vi "RDC-tools-generate_temp_array.vi"(7 "Increment":dbl=0.1, 11 "temp Cx10":dbl[](array[numeric])) -> (3 "temp C":dbl[](array[numeric]))   [LabVIEW 2020, in "RDC-Reflection_Data_Computation.lvlib"]
doc: "Generates an evenly spaced temperature array that runs from the first to the last element of the input array in steps of Increment. Used by the water and salt water generate_parameter VIs to build the temperatures the model parameters are interpolated at."
uses:
  RDC-Reflection_Data_Computation.lvlib
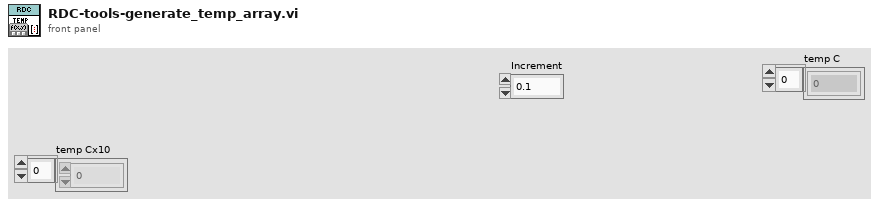
[diagram p1: front panel]
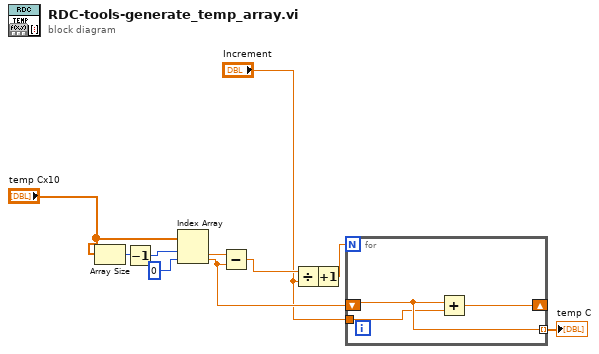
[diagram p0: block diagram]
diagram:
  n1 = Array Size(array="temp Cx10") -> (size(s)=w7:i32)
  n2 = Decrement(x=w7) -> (x-1=w11:i32)
  n3 = Index Array(array="temp Cx10", index #1=w11, index #2=0 ("index")) -> (element #1=w9:dbl, element #2=w8:dbl)
  n4 = Subtract(x=w9, y=w8) -> (x-y=w5:dbl)
  n5 = Divide(x=w5, y="Increment") -> (x/y=w6:dbl)
  n6 = Increment(x=w6) -> (x+1=w4:dbl)
  n7 = for {
    N: w4 -> [_]
    tunnel: [w14] -> w3 mode=indexing
    shift-right: [w13] -> _
    shift-left: w8 -> [w14]
    tunnel: "Increment" -> [w12]
    n8 = Add(x=w14, y=w12) -> (x+y=w13:dbl)
  }
  "temp C" <- w3
